vi "Read Phase.vi"(8 "error in (no error)":errorcluster, 11 "Sequence Executor in":refnum<class "Sequence Executor.lvclass">) -> (0 "error out":errorcluster, 2 "Step Phase":T1, 3 "Sequence Executor out":refnum<class "Sequence Executor.lvclass">)   [LabVIEW 2026, in "Sequence Executor.lvclass"]
doc: "Reads one field of this class's private data. Generated by lvai_create_accessors from the class private data control."
uses:
  Sequence Executor.lvclass
  Typedefs/Step Phase.ctl
  Sequence Executor.lvclass/Sequence Executor.ctl
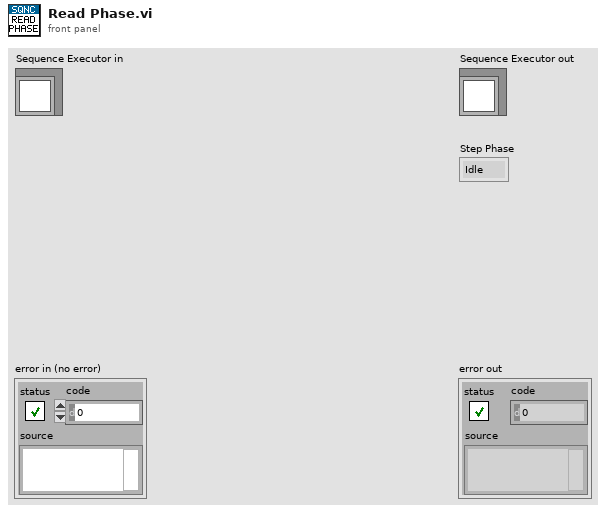
[diagram p1: front panel]
types:
  T1 = typedef "Step Phase.ctl" = enum16{"Idle", "Settling", "Dwell", "Complete"}
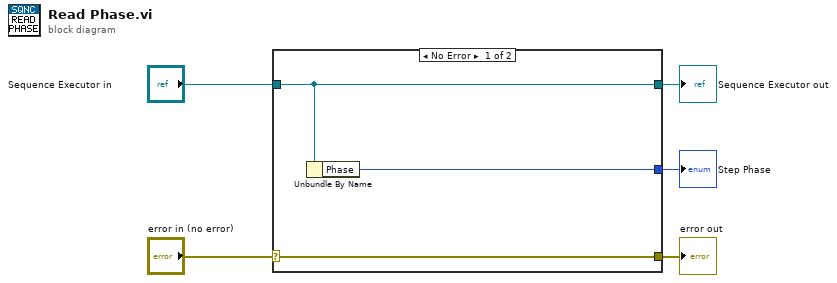
[diagram p0: block diagram]
diagram:
  n1 = case shown="No Error" "error in (no error)" {
    selector: "error in (no error)" -> [w8 w9]
    tunnel: [w8 w9] -> w4
    tunnel: [w7 w10] -> w2
    tunnel: "Sequence Executor in" -> [w7 w10]
    tunnel: [w6 _] -> w1
    frame No Error {
      n2 = Unbundle By Name(w7) -> ("Phase"=w6:T1)
    }
    frame Error {
    }
  }
  "error out" <- w4
  "Sequence Executor out" <- w2
  "Step Phase" <- w1
